vi "FunctionGenerator_Add_Value.vi"(9 "Y Value":dbl, 10 "X Value":dbl, 11 "in FUNCTION_GENERATOR":T1) -> (3 "out FUNCTION_GENERATOR":T1)   [LabVIEW 2019, in "Trajectory_Library.lvlib"]
doc: "Insert new X, Y pair into an existing Function Generator data cluster. If the X values matches an existing X value, the new X and Y values replaces the old values.\n\nInputs:\n - In Function Generator -- Function generator data cluster\n - X -- X value\n - Y -- Y value\n\nOutputs:\n - out Function Generator -- updated data structure"
uses:
  Trajectory_Library.lvlib
  TypeDef/FUNCTION_GENERATOR.ctl
  <vilib>/gmath/NI_Gmath.lvlib
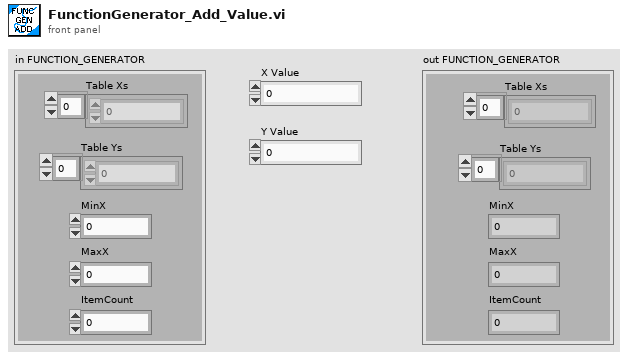
[diagram p1: front panel]
types:
  T1 = typedef "Trajectory_Library.lvlib/FUNCTION_GENERATOR.ctl" = cluster{"Table Xs":dbl[], "Table Ys":dbl[], "MinX":dbl, "MaxX":dbl, "ItemCount":i32}
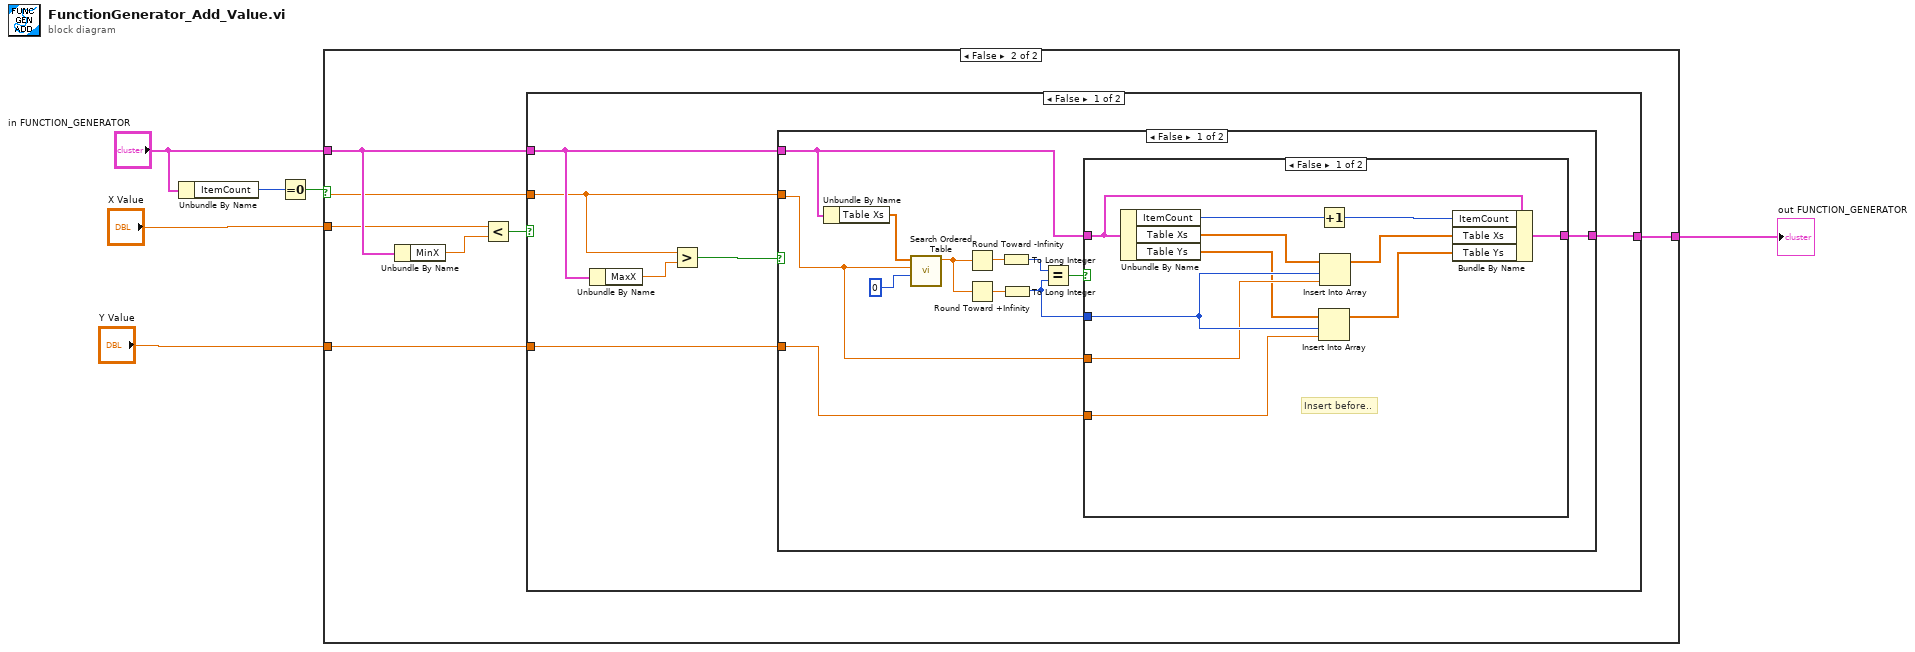
[diagram p0: block diagram]
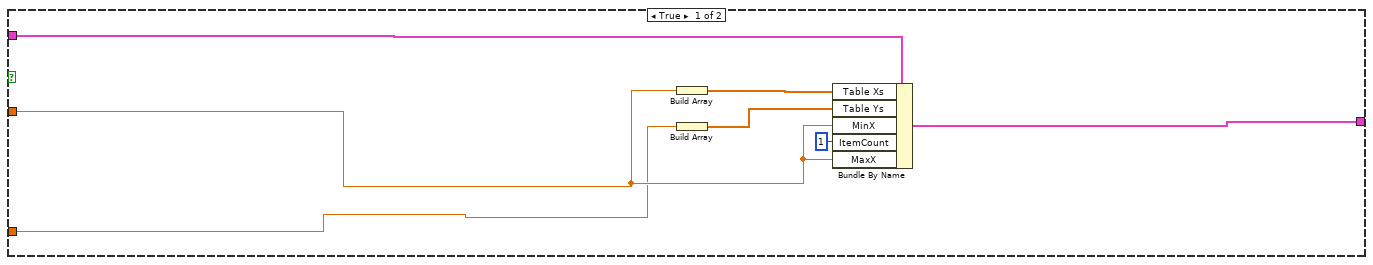
[diagram p2: hidden frame]
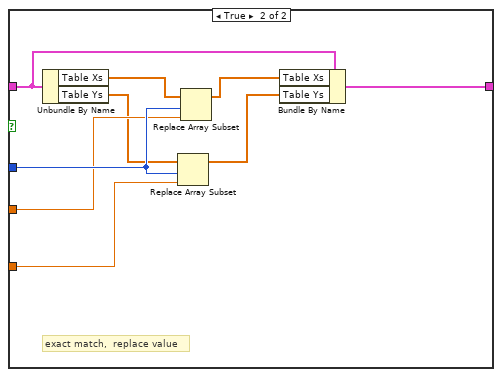
[diagram p3: hidden frame]
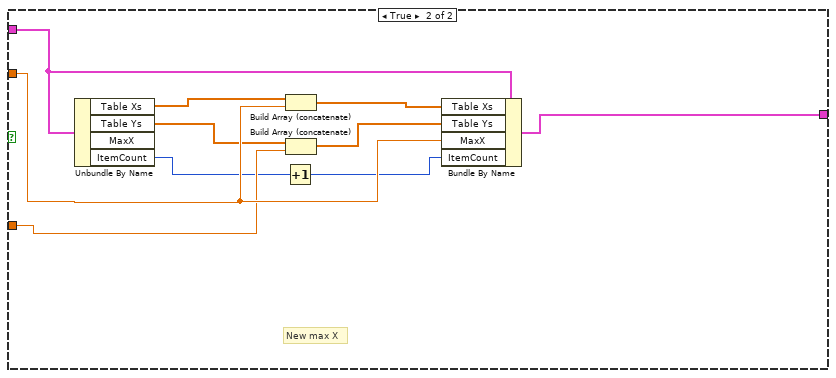
[diagram p4: hidden frame]
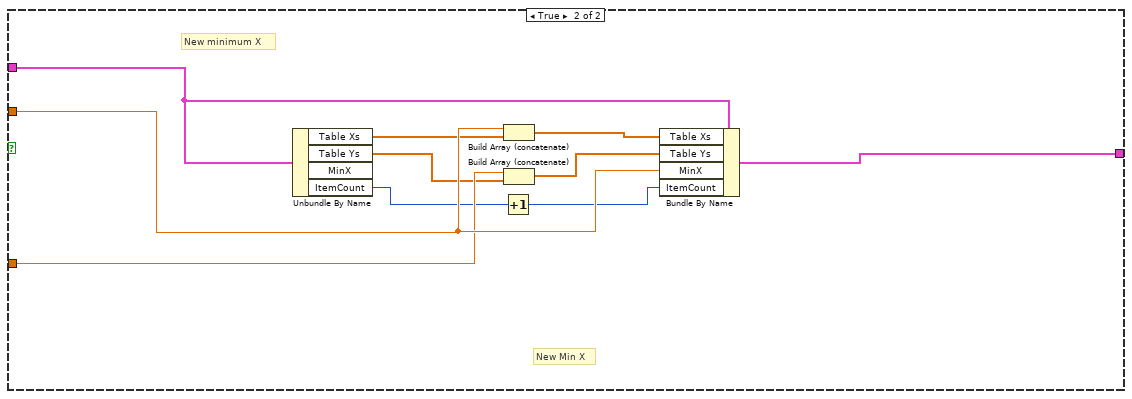
[diagram p5: hidden frame]
diagram:
  n1 = Unbundle By Name("in FUNCTION_GENERATOR") -> ("ItemCount"=w1:i32)
  n2 = Equal To 0?(x=w1) -> (x = 0?=w2:bool)
  n3 = case shown="False" w2 {
    tunnel: "in FUNCTION_GENERATOR" -> [w13 w17]
    tunnel: "X Value" -> [w11 w16]
    tunnel: "Y Value" -> [w10 w15]
    tunnel: [w12 w14] -> w4
    frame True {
      n4 = Build Array(w11) -> (w9:dbl[])
      n5 = Build Array(w10) -> (w8:dbl[])
      n6 = Bundle By Name(cluster=w13, "Table Xs"=w9, "Table Ys"=w8, "MinX"=w11, "ItemCount"=1, "MaxX"=w11) -> (w12:T1)
    }
    frame False {
      n7 = Unbundle By Name(w17) -> ("MinX"=w19:dbl)
      n8 = Less?(x=w16, y=w19) -> (x < y?=w18:bool)
      n9 = case shown="False" w18 {
        tunnel: w17 -> [w24 w77]
        tunnel: w16 -> [w22 w76]
        tunnel: w15 -> [w21 w75]
        tunnel: [w23 w74] -> w14
        frame False {
          n10 = Unbundle By Name(w24) -> ("MaxX"=w25:dbl)
          n11 = Greater?(x=w22, y=w25) -> (0:w20:bool)
          n12 = case shown="False" w20 {
            tunnel: w24 -> [w30 w67]
            tunnel: [w26 w66] -> w23
            tunnel: w22 -> [w28 w65]
            tunnel: w21 -> [w27 w64]
            frame False {
              n13 = Unbundle By Name(w30) -> ("Table Xs"=w36:dbl[])
              n14 = call <vilib>:"Search Ordered Table.vi"("starting index"=0, "x value"=w28, "ordered x array"=w36) -> ("fractional index"=w35:dbl)  [unwired: 8 in]
              n15 = Round Toward -Infinity(1:w35) -> (0:w33:dbl)
              n16 = Round Toward +Infinity(x=w35) -> (ceil(x): smallest int >= x=w34:dbl)
              n17 = To Long Integer(number=w33) -> (32bit integer=w32:i32)
              n18 = To Long Integer(number=w34) -> (32bit integer=w29:i32)
              n19 = Equal?(x=w32, y=w29) -> (x = y?=w31:bool)
              n20 = case shown="False" w31 {
                tunnel: w30 -> [w45 w57]
                tunnel: w29 -> [w48 w56]
                tunnel: w28 -> [w47 w55]
                tunnel: w27 -> [w46 w54]
                tunnel: [w44 w53] -> w26
                frame False {
                  # "Insert before.."
                  n21 = Unbundle By Name(w45) -> ("ItemCount"=w43:i32, "Table Xs"=w41:dbl[], "Table Ys"=w40:dbl[])
                  n22 = Increment(x=w43) -> (x+1=w42:i32)
                  n23 = Insert Into Array(array=w40, index=w48, new element=w46) -> (w38:dbl[])
                  n24 = Insert Into Array(array=w41, index=w48, new element=w47) -> (w39:dbl[])
                  n25 = Bundle By Name(cluster=w45, "ItemCount"=w42, "Table Xs"=w39, "Table Ys"=w38) -> (w44:T1)
                }
                frame True {
                  # "exact match,  replace value"
                  n26 = Unbundle By Name(w57) -> ("Table Xs"=w52:dbl[], "Table Ys"=w51:dbl[])
                  n27 = Replace Array Subset(array=w51, new element=w54, index=w56) -> (w49:dbl[])
                  n28 = Replace Array Subset(array=w52, new element=w55, index=w56) -> (w50:dbl[])
                  n29 = Bundle By Name(cluster=w57, "Table Xs"=w50, "Table Ys"=w49) -> (w53:T1)
                }
              }
            }
            frame True {
              # "New max X"
              n30 = Unbundle By Name(w67) -> ("Table Xs"=w59:dbl[], "Table Ys"=w58:dbl[], "ItemCount"=w61:i32)  [unwired: 1 out]
              n31 = Increment(x=w61) -> (x+1=w60:i32)
              n32 = Build Array (concatenate)(w59, w65) -> (w63:dbl[])
              n33 = Build Array (concatenate)(w58, w64) -> (w62:dbl[])
              n34 = Bundle By Name(cluster=w67, "Table Xs"=w63, "Table Ys"=w62, "MaxX"=w65, "ItemCount"=w60) -> (w66:T1)
            }
          }
        }
        frame True {
          # "New Min X"
          # "New minimum X"
          n35 = Unbundle By Name(w77) -> ("Table Xs"=w73:dbl[], "Table Ys"=w70:dbl[], "ItemCount"=w69:i32)  [unwired: 1 out]
          n36 = Increment(x=w69) -> (x+1=w68:i32)
          n37 = Build Array (concatenate)(w76, w73) -> (w72:dbl[])
          n38 = Build Array (concatenate)(w75, w70) -> (w71:dbl[])
          n39 = Bundle By Name(cluster=w77, "Table Xs"=w72, "Table Ys"=w71, "MinX"=w76, "ItemCount"=w68) -> (w74:T1)
        }
      }
    }
  }
  "out FUNCTION_GENERATOR" <- w4
